vi "MQTT Client - Read.vi"(0 "MQTT Session":T2, 7 "timeout (global)":i32=10, 11 "error in (no error)":errorcluster) -> (2 "# received":u64, 4 "MQTT Session out":T2, 6 "Topic":string, 8 "Message":string, 10 "New message?":bool, 14 "Publish Properties Received (V5)":T1[](array[typedef]) {"Property" items=[" Payload Format Indicator          "=1, " Message Expiry Interval           "=2, " Content Type                      "=3, " Response Topic                    "=8, " Correlation Data                  "=9, " Subscription Identifier           "=11, " Topic Alias                       "=35, " User Property                     "=38]}, 15 "error out":errorcluster)   [LabVIEW 2019, in "KoRE-MQTT.lvlib"]
doc: "<b>Description:</b> This VI manages the core reading operations of the MQTT client by continuously checking for incoming messages from the broker. It handles message reception while maintaining the MQTT session, integrating Quality of Service (QoS) features, and facilitating message processing.\n\n<b>Input Terminals:</b>\n- <b>MQTT Session [0]</b>: Reference to the active MQTT session that allows communication with the broker.\n- <b>timeout (global) [7]</b>: Time interval in seconds for waiting for incoming messages before timing out.\n\n<b>Output Terminals:</b>\n- <b># received [2]</b>: Number of messages received from the broker during the execution of this VI.\n- <b>MQTT Session out [4]</b>: Reference to the active MQTT session after processing the read operation.\n- <b>Topic [6]</b>: The topic associated with the last received message, provided only when \"New message?\" is true.\n- <b>Message [8]</b>: The content of the last message that was received, provided only when \"New message?\" is true.\n- <b>New message? [10]</b>: Boolean value indicating whether a new message has been received since the last iteration. If false, no new messages are available, or the VI is busy handling subscriptions or QoS.\n- <b>Publish Properties [14]</b>: Array of properties associated with the last message received, applicable only for MQTT v5 connections, provided only when \"New message?\" is true.\n\n\nCopyright (c) 2025 KoRElibs.com\nSPDX-License-Identifier: EUPL-1.2\n\nThis VI is licensed under the European Union Public License (EUPL) Version 1.2. You may use this VI unmodified in proprietary works. If you distribute a modified version of this file, the modified file must be released under the EUPL-1.2. Full license: https://joinup.ec.europa.eu/asset/eupl/eupl/1.2/"
uses:
  KoRE-MQTT.lvlib
  TypeDefs/MQTT Client Session.ctl
  TypeDefs/MQTT Property - PUBLISH.ctl
  TypeDefs/MQTT Property Type.ctl
  Private/TypeDefs/MQTT Packet - Type.ctl
  Private/TypeDefs/MQTT Client Session - Data Value Reference.ctl
  TypeDefs/MQTT Client Session - Data.ctl
  TypeDefs/MQTT Property - Will.ctl
  TypeDefs/MQTT Property - CONNECT.ctl
  Private/TypeDefs/MQTT Subscription - Info.ctl
  Private/MQTT Session - Get TCP Info.vi
  Private/MQTT Session - Reset Keep Alive Timer.vi
  Private/MQTT Data Stream - Write Packet.vi
  Private/MQTT Data - Encode Varint.vi
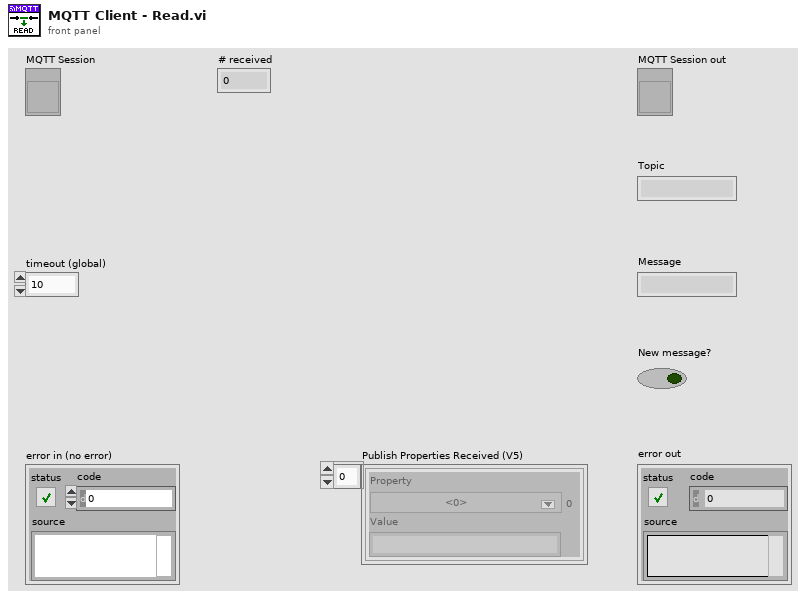
[diagram p1: front panel]
types:
  T1 = typedef "KoRE-MQTT.lvlib/MQTT Property - PUBLISH.ctl" = cluster{"Property":u8, "Value":string}
  T2 = typedef "KoRE-MQTT.lvlib/MQTT Client Session.ctl" = refnum<vi>
  T3 = typedef "KoRE-MQTT.lvlib/MQTT Packet - Type.ctl" = enum32{"Reserved", "CONNECT", "CONNACK", "PUBLISH", "PUBACK", "PUBREC", "PUBREL", "PUBCOMP", "SUBSCRIBE", "SUBACK", "UNSUBSCRIBE", "UNSUBACK", "PINGREQ", "PINGRESP", "DISCONNECT", "AUTH"}
  T4 = typedef "KoRE-MQTT.lvlib/MQTT Client Session - Data Value Reference.ctl" = refnum<data-value>
  T5 = typedef "KoRE-MQTT.lvlib/MQTT Packet - Fixed Header.ctl" = cluster{"MessageType":T3, "DUP Flag":bool, "QoS Level":u8, "RETAIN":bool, "Remaining Length":u32}
  T6 = typedef "KoRE-MQTT.lvlib/MQTT Property Type.ctl" = u8
  T7 = typedef "KoRE-MQTT.lvlib/MQTT Property - GENERIC.ctl" = cluster{"Property":T6, "Value":string}
  T8 = typedef "KoRE-MQTT.lvlib/MQTT Client Session - Data.ctl" = cluster{"TCP ref":refnum<k5>, "Next Packet Id":u16, "Version":u8, "Host":string, "Port":u16, "Ping Delta":u32, "Username":string, "Password":string, "Will QoS":u8, "Will Retain":bool, "Will Topic":string, "Will Payload":string, "TCP Timeout":i32, "Semaphore":T9, "In-Flight Messages":variant, "Close":bool, "Last Send":u32, "Keep Alive":u16, "Last Ping RTT":u32, "Last Ping":u32, "Will Properties":T10[], "Session Expiry Interval":u32, "Maximum QoS":u8, "Retain Available":bool, "Server Maximum Packet Size":u32, "Client Identifier":string, "Server Topic Alias Maximum":u16, "Wildcard Subscription Available":bool, "Subscription Identifier Available":bool, "Shared Subscription Available":bool, "Connect Properties":T11[], "Client Maximum Packet Size":u32, "Client Topic Alias Maximum":u16, "Server Receive Maximum":u16, "Client Receive Maximum":u16, "TLS cfg":refnum<k36>, "Subscriptions":T12[]}
  T9 = typedef "Semaphore RefNum" = refnum<k1>
  T10 = typedef "KoRE-MQTT.lvlib/MQTT Property - Will.ctl" = cluster{"Property":u8, "Value":string}
  T11 = typedef "KoRE-MQTT.lvlib/MQTT Property - CONNECT.ctl" = cluster{"Property":u8, "Value":string}
  T12 = typedef "KoRE-MQTT.lvlib/MQTT Subscription - Info.ctl" = cluster{"Packet Id":u16, "Index":u16, "Identifier":u32, "QoS":u8, "Topic Filter":string, "Reason Code":u8, "Reason String":string, "Granted":bool}
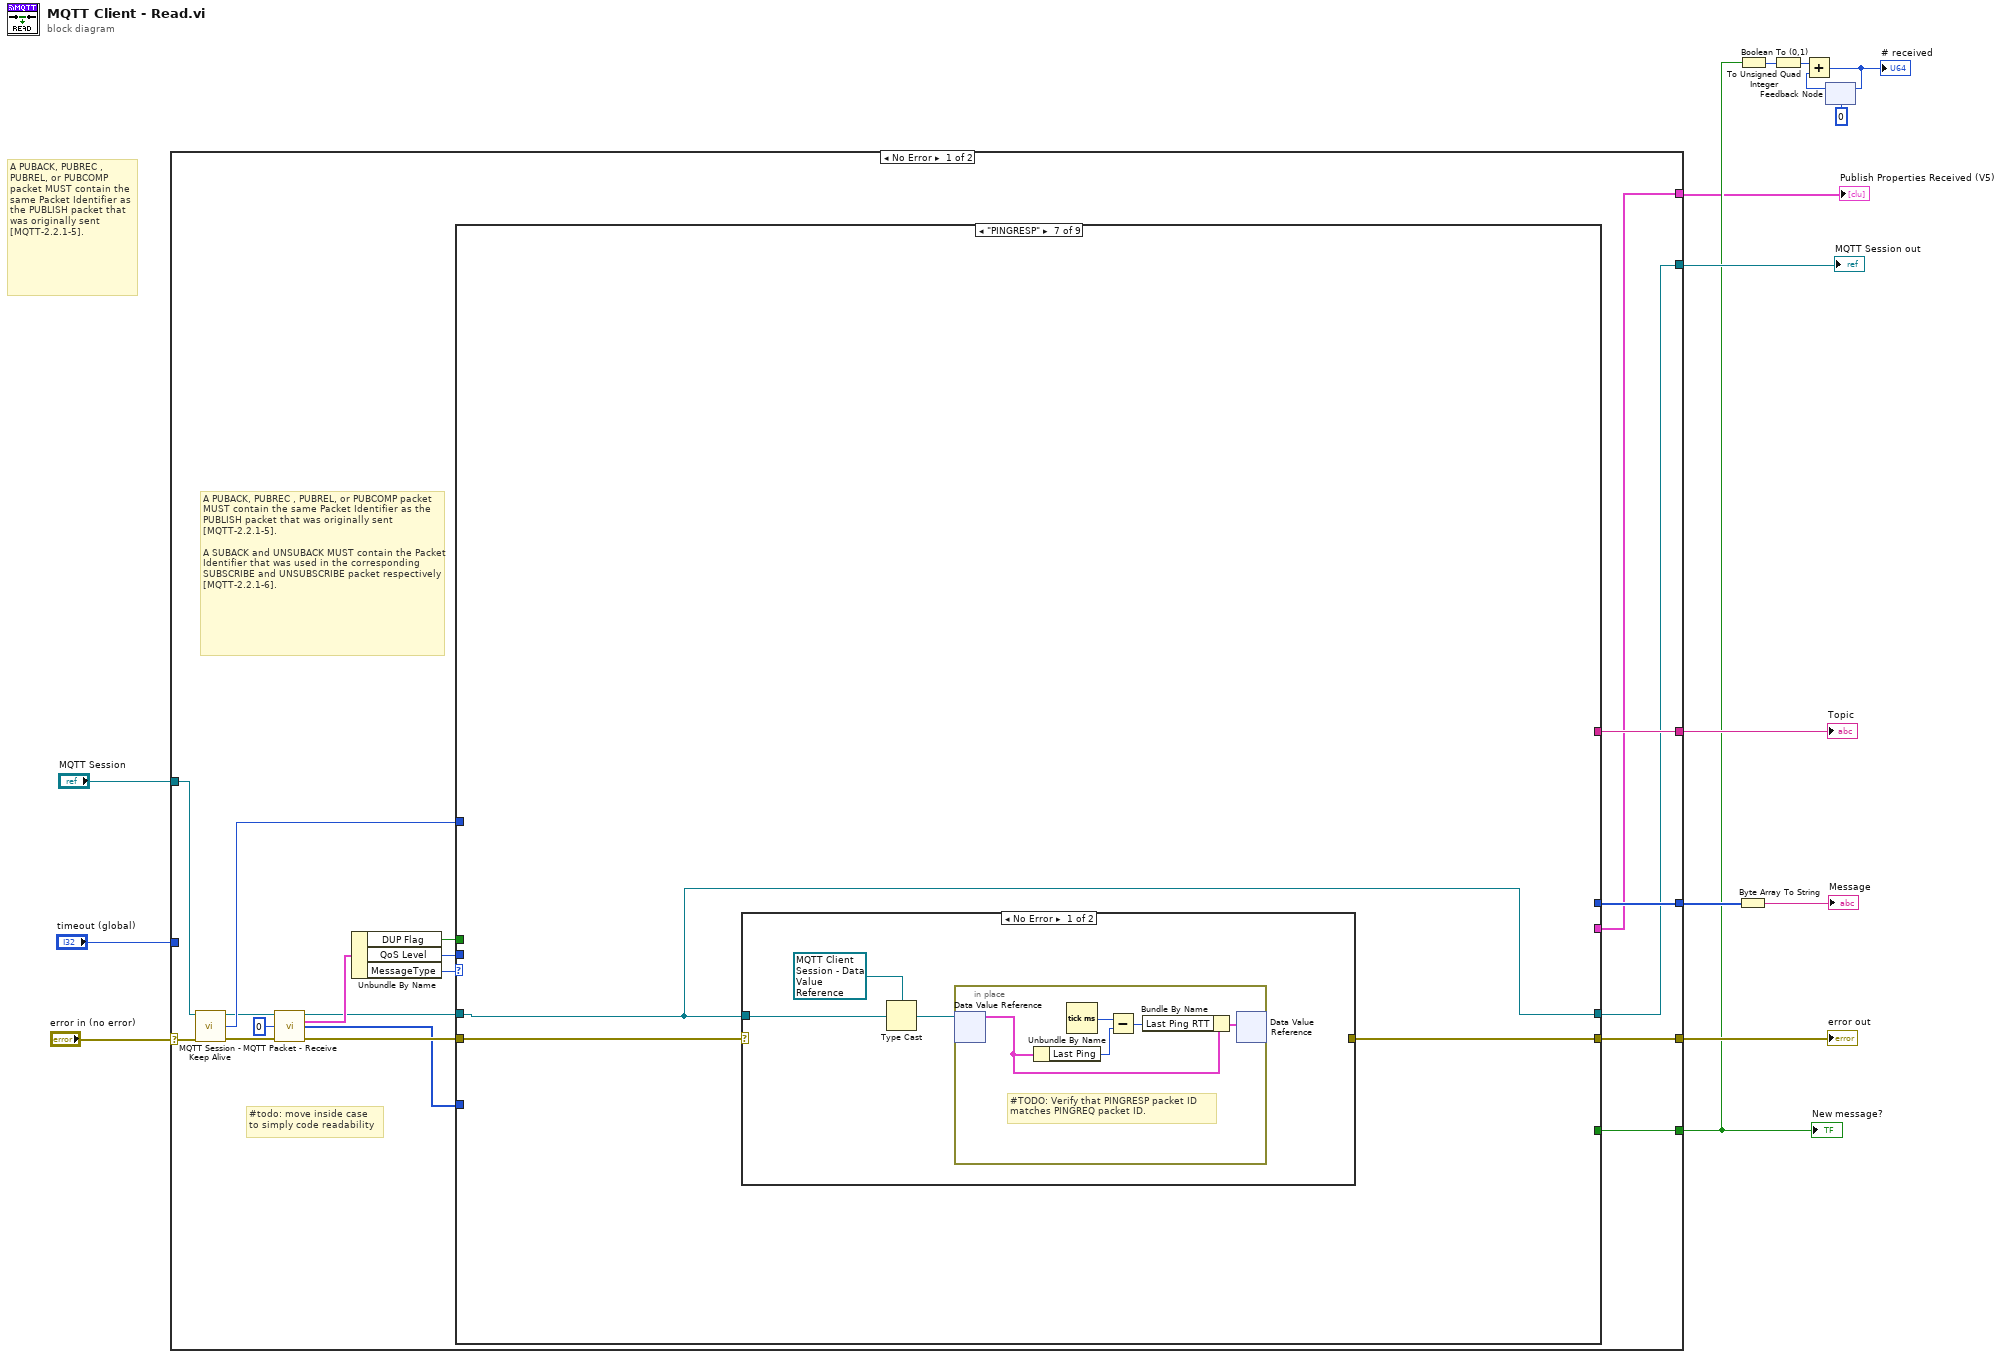
[diagram p0: block diagram]
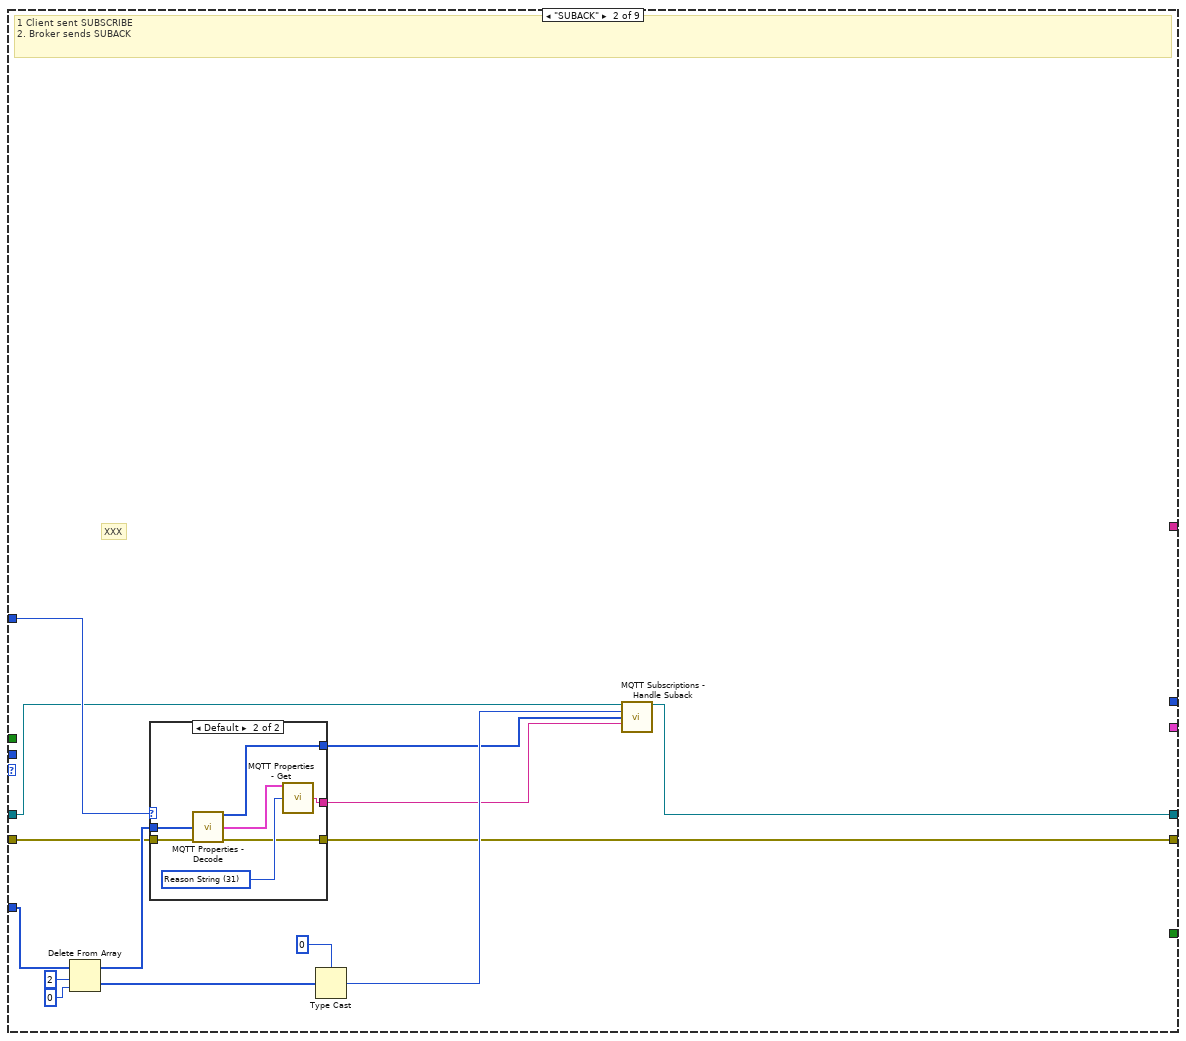
[diagram p3: hidden frame]
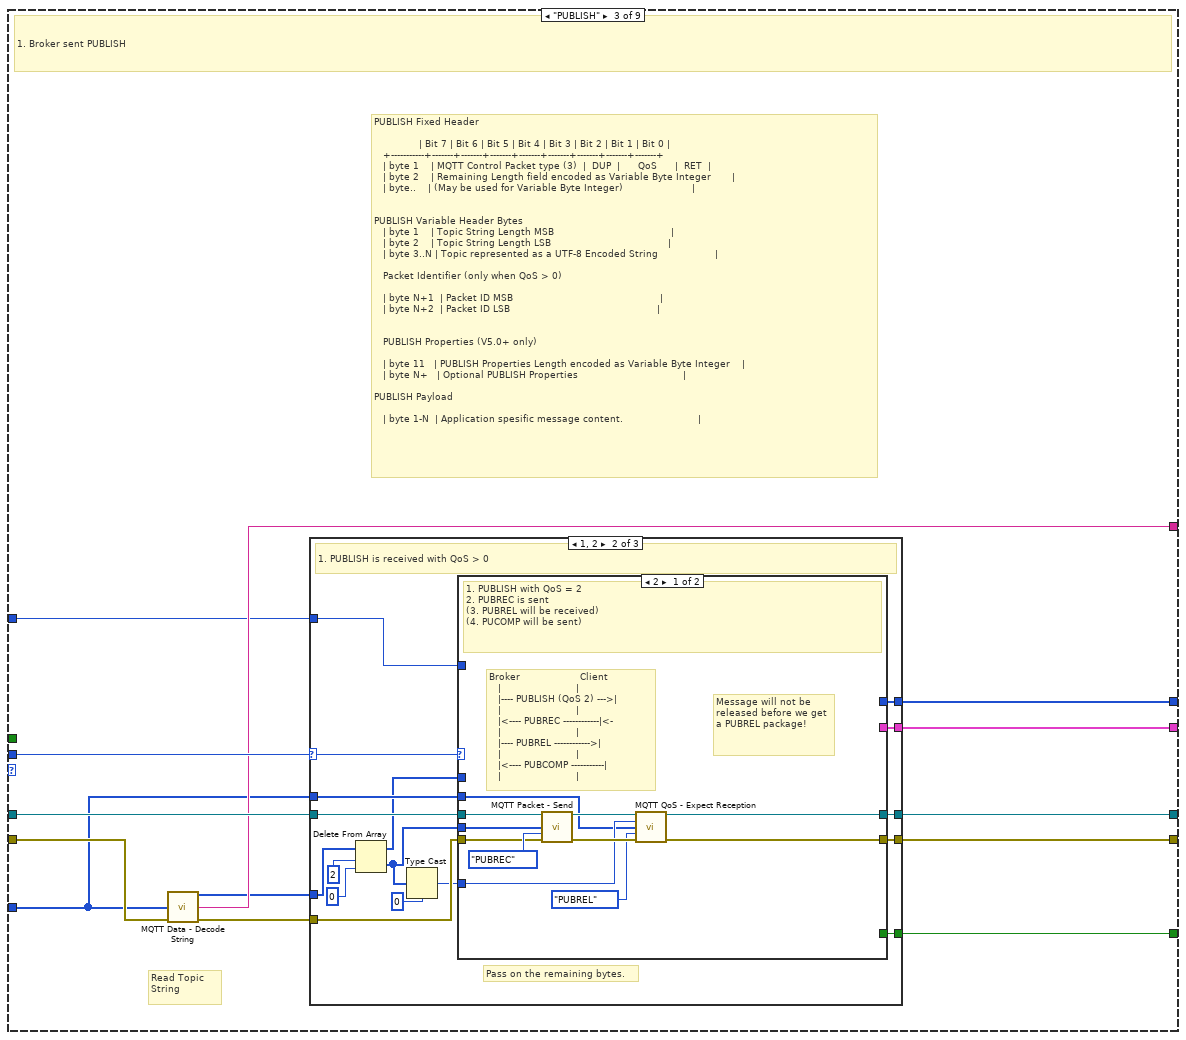
[diagram p5: hidden frame]
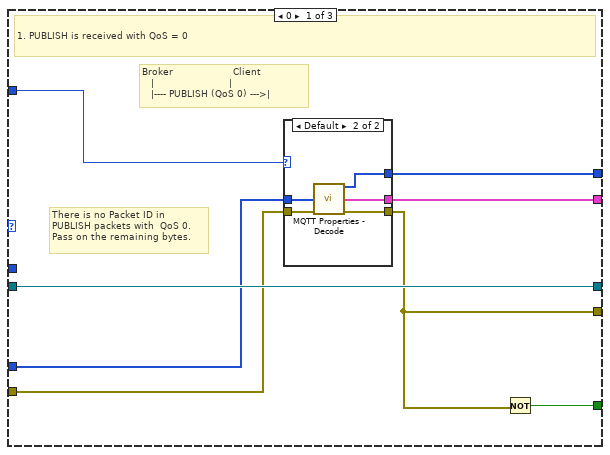
[diagram p6: hidden frame]
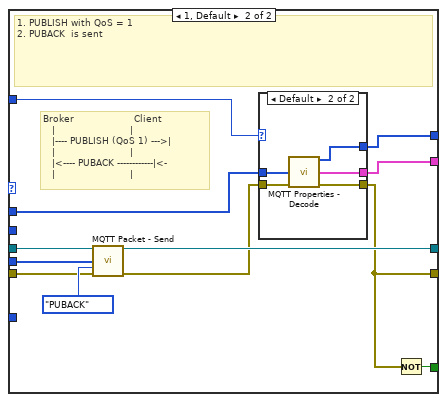
[diagram p8: hidden frame]
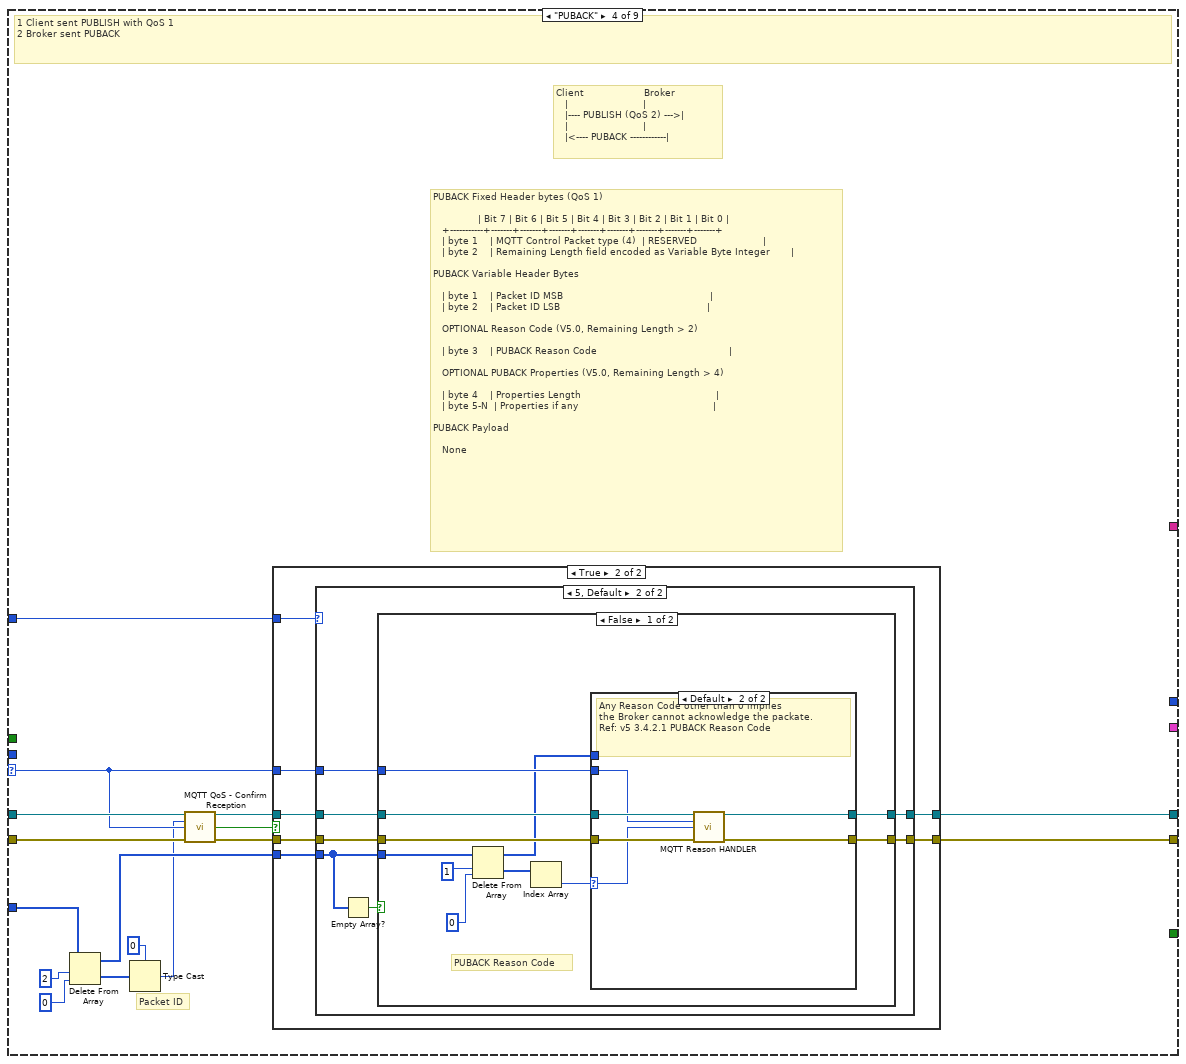
[diagram p11: hidden frame]
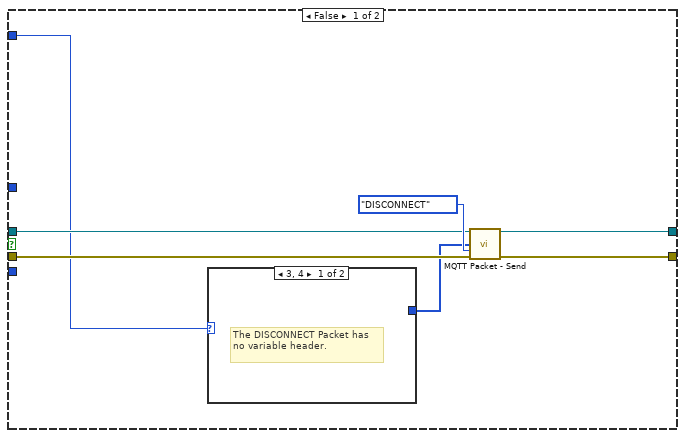
[diagram p12: hidden frame]
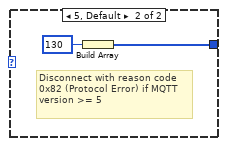
[diagram p13: hidden frame]
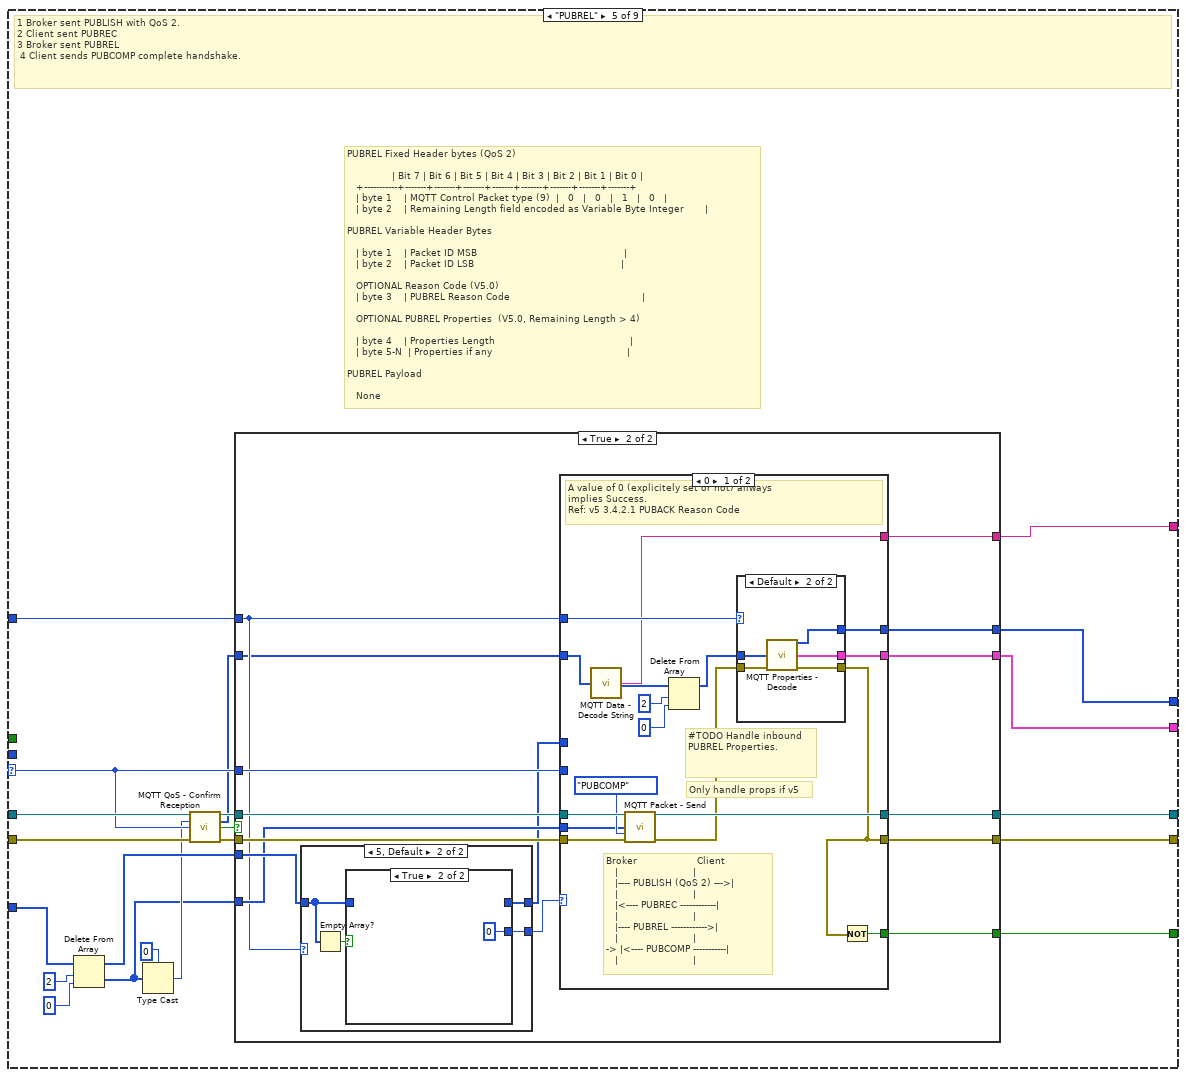
[diagram p17: hidden frame]
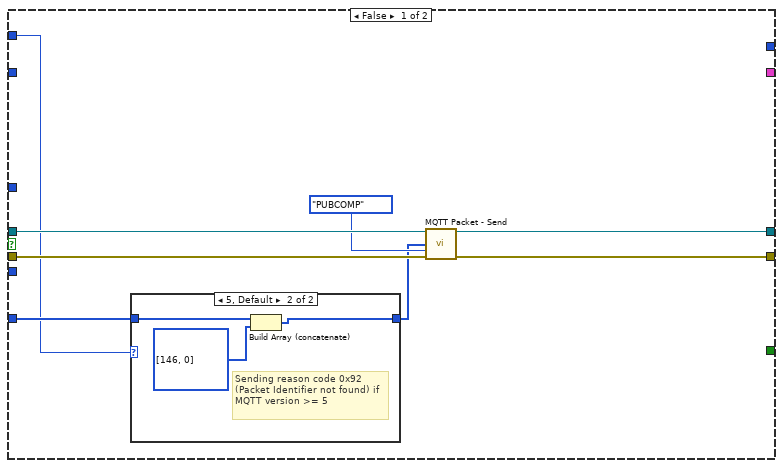
[diagram p18: hidden frame]
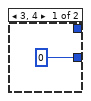
[diagram p20: hidden frame]
diagram:
  # "A PUBACK, PUBREC , PUBREL, or PUBCOMP packet MUST contain the same Packet Identifier as the PUBLISH packet that was originally sent [MQTT-2.2.1-5]."
  n1 = case shown="No Error" "error in (no error)" {
    selector: "error in (no error)" -> [w31 w387]
    tunnel: [w25 w387] -> w14
    tunnel: "MQTT Session" -> [w19 w386]
    tunnel: [w24 w386] -> w12
    tunnel: "timeout (global)" -> [_ _]
    tunnel: [w34 _] -> w10
    tunnel: [w33 _] -> w8
    tunnel: [w23 _] -> w4
    tunnel: [w21 _] -> w1
    frame No Error {
      # "#todo: move inside case \nto simply code readability"
      # "A PUBACK, PUBREC , PUBREL, or PUBCOMP packet MUST contain the same Packet Identifier as the PUBLISH packet that was originally sent [MQTT-2.2.1-5].\n\nA SUBACK and UNSUBACK MUST contain the Packet Identifier that was used in the corresponding SUBSCRIBE and UNSUBSCRIBE packet respectively [MQTT-2.2.1-6]."
      n2 = call "MQTT Session - Keep Alive.vi"("mqtt ref in"=w19, "error in"=w31) -> ("mqtt ref out"=w28:T2, "Version"=w32:u8, "error out"=w29:errorcluster)  [unwired: 11 in]
      n3 = call "MQTT Packet - Receive.vi"("mqtt ref in"=w28, "timeout (global)"=0, "error in"=w29) -> ("mqtt ref out"=w18:T2, "Fixed Header"=w30:T5, "Remaining Data"=w16:u8[], "error out"=w17:errorcluster)  [unwired: 7 in, 2 out]
      n4 = Unbundle By Name(w30) -> ("DUP Flag"=w26:bool, "QoS Level"=w27:u8, "MessageType"=w22:T3)
      n5 = case shown="\"PINGRESP\"" w22 {
        selector: w22 -> [_ _ _ w140 w207 w300 _ _ w363]
        tunnel: w27 -> [_ _ w72 _ _ _ _ _ _]
        tunnel: w32 -> [_ w50 w65 w150 w218 w294 _ w346 w364]
        tunnel: [_ _ w70 _ w198 _ _ _ _] -> w34
        tunnel: [_ _ w64 _ w201 _ _ _ _] -> w33
        tunnel: w18 -> [w36 w38 w71 w145 w213 w298 w326 w337 w368]
        tunnel: w17 -> [w35 w39 w68 w144 w211 w299 w327 w338 w369]
        tunnel: [w36 w46 w62 w152 w217 w292 w326 w347 w374] -> w24
        tunnel: [w35 w37 w61 w151 w216 w291 w325 w340 w373] -> w25
        tunnel: w26 -> [_ _ _ _ _ _ _ _ _]
        tunnel: [_ _ w66 _ w199 _ _ _ _] -> w23
        tunnel: w16 -> [_ w42 w60 w147 w208 w293 _ w343 w370]
        tunnel: [_ _ w63 _ w200 _ _ _ _] -> w21
        frame Default {
          # "#TODO:  Handle reading of unknown/unsupported MQTT Packet types, e.i. log / error handling."
        }
        frame "SUBACK" {
          # "XXX"
          # "1 Client sent SUBSCRIBE\n2. Broker sends SUBACK"
          n6 = Delete From Array(array=w42, length=2, index=0) -> (deleted portion=w40:u8[], array with subset deleted=w41:u8[])
          n7 = case shown="Default" w50 {
            tunnel: [w52 w59] -> w47
            tunnel: w41 -> [w52 w58]
            tunnel: [_ w56] -> w45
            tunnel: w39 -> [w51 w54]
            tunnel: [w51 w53] -> w37
            frame 3, 4 {
            }
            frame Default {
              w55 = T6 31 items=["Payload Format Indicator"=1, "Message Expiry Interval"=2, "Content Type"=3, "Response Topic"=8, "Correlation Data"=9, "Subscription Identifier"=11, "Session Expiry Interval"=17, "Assigned Client Identifier"=18, "Server Keep Alive"=19, "Authentication Method"=21, "Authentication Data"=22, "Request Problem Information"=23, "Will Delay Interval"=24, "Request Response Information"=25, "Response Information"=26, "Server Reference"=28, "Reason String"=31, "Receive Maximum"=33, "Topic Alias Maximum"=34, "Topic Alias"=35, "Maximum QoS"=36, "Retain Available"=37, "User Property"=38, "Maximum Packet Size"=39, "Wildcard Subscription Available"=40, "Subscription Identifier Available"=41, "Shared Subscription Available"=42] ("MQTT Property Type")
              n8 = call "MQTT Properties - Decode.vi"("Encoded MQTT Properties"=w58, "error in (no error)"=w54) -> ("remaining data"=w59:u8[], "MQTT Properties"=w57:T7[], "error out"=w53:errorcluster)  [unwired: 11 in]
              n9 = call "MQTT Properties - Get.vi"("MQTT Properties"=w57, "MQTT Property Type"=w55) -> ("Value"=w56:string)  [unwired: 11 in, 2 out]
            }
          }
          n10 = Type Cast(type=u16 0, x=w40) -> (*(type *) &x=w48:u16)
          n11 = call "MQTT Subscriptions - Handle Suback.vi"("MQTT ref in"=w38, "Packet ID"=w48, "Reason Codes"=w47, "Reason String"=w45) -> ("MQTT ref out"=w46:T2)  [unwired: 11 in]
        }
        frame "PUBLISH" {
          # "PUBLISH Fixed Header\n\n               | Bit 7 | Bit 6 | Bit 5 | Bit 4 | Bit 3 | Bit 2 | Bit 1 | Bit 0 |\n   +-----------+-------+-------+-------+-------+-------+-------+-------+-------+\n   | byte 1    | MQTT Control Packet type (3)  |  DUP  |      QoS      |  RET  |\n   | byte 2    | Remaining Length field encoded as Variable Byte Integer       |\n   | byte..    | (May be used for Variable Byte Integer)                       | \n\n\nPUBLISH Variable Header Bytes\n   | byte 1    | Topic String Length MSB                                       |  \n   | byte 2    | Topic String Length LSB                                       |  \n   | byte 3..N | Topic represented as a UTF-8 Encoded String                   |\n\n   Packet Identifier (only when QoS > 0)   \n\n   | byte N+1  | Packet ID MSB                                                 |  \n   | byte N+2  | Packet ID LSB                                                 |\n\n\n   PUBLISH Properties (V5.0+ only)\n\n   | byte 11   | PUBLISH Properties Length encoded as Variable Byte Integer    |\n   | byte N+   | Optional PUBLISH Properties                                   |\n\nPUBLISH Payload \n\n   | byte 1-N  | Application spesific message content.                         |"
          # "Read Topic String"
          # "1. Broker sent PUBLISH"
          n12 = call "MQTT Data - Decode String.vi"("Encoded String"=w60, "error in (no error)"=w68) -> ("remaining data"=w69:u8[], "String"=w70:string, "error out"=w67:errorcluster)  [unwired: 11 in]
          n13 = case shown="1, 2" w72 {
            selector: w72 -> [_ w102 _]
            tunnel: w69 -> [w78 w97 _]
            tunnel: w71 -> [w80 w101 w136]
            tunnel: w67 -> [w75 w100 w135]
            tunnel: [w73 w99 w135] -> w61
            tunnel: [w80 w98 w136] -> w62
            tunnel: [w79 w89 _] -> w66
            tunnel: [w77 w91 _] -> w64
            tunnel: [w76 w90 _] -> w63
            tunnel: w65 -> [w74 w92 _]
            tunnel: w60 -> [_ w93 _]
            frame 0 {
              # "There is no Packet ID in\nPUBLISH packets with  QoS 0.\nPass on the remaining bytes."
              # "Broker                    Client\n   |                         |\n   |---- PUBLISH (QoS 0) --->|"
              # "1. PUBLISH is received with QoS = 0"
              n14 = case shown="Default" w74 {
                tunnel: w78 -> [w82 w87]
                tunnel: [w82 w86] -> w77
                tunnel: [_ w85] -> w76
                tunnel: w75 -> [w81 w84]
                tunnel: [w81 w83] -> w73
                frame 3, 4 {
                }
                frame Default {
                  n15 = call "MQTT Properties - Decode.vi"("Encoded MQTT Properties"=w87, "error in (no error)"=w84) -> ("remaining data"=w86:u8[], "MQTT Properties"=w85:T7[], "error out"=w83:errorcluster)  [unwired: 11 in]
                }
              }
              n16 = Not(x=w73) -> (.not. x?=w79:bool)
            }
            frame 1, 2 {
              # "Pass on the remaining bytes."
              # "1. PUBLISH is received with QoS > 0"
              n17 = Delete From Array(array=w97, length=2, index=0) -> (deleted portion=w94:u8[], array with subset deleted=w88:u8[])
              n18 = Type Cast(type=u16 0, x=w94) -> (*(type *) &x=w95:u16)
              n19 = case shown="2" w102 {
                tunnel: w95 -> [w108 _]
                tunnel: w101 -> [w114 w126]
                tunnel: [w109 w125] -> w98
                tunnel: w100 -> [w113 w124]
                tunnel: [w111 w117] -> w99
                tunnel: w94 -> [w106 w123]
                tunnel: w93 -> [w105 _]
                tunnel: w92 -> [_ w122]
                tunnel: [_ w121] -> w91
                tunnel: [_ w119] -> w90
                tunnel: [_ w118] -> w89
                tunnel: w88 -> [_ w116]
                frame 2 {
                  # "Message will not be released before we get a PUBREL package!"
                  # "Broker                    Client\n   |                         |\n   |---- PUBLISH (QoS 2) --->|\n   |                         |\n   |<---- PUBREC ------------|<-\n   |                         |\n   |---- PUBREL ------------>|\n   |                         |\n   |<---- PUBCOMP -----------|\n   |                         |"
                  # "1. PUBLISH with QoS = 2\n2. PUBREC is sent\n(3. PUBREL will be received)\n(4. PUCOMP will be sent)"
                  n20 = call "MQTT Packet - Send.vi"("mqtt ref in"=w114, "packet data"=w106, "MessageType"=MQTT_Packet_-_Type."PUBREC", "error in (no error)"=w113) -> ("mqtt ref out"=w110:T2, "error out"=w112:errorcluster)  [unwired: 9 in, 1 out]
                  n21 = call "MQTT QoS - Expect Reception.vi"("MQTT Reference"=w110, "Packet ID"=w108, "Message"=w105, "MessageType"=MQTT_Packet_-_Type."PUBREL", "Error In"=w112) -> ("MQTT Reference"=w109:T2, "Error Out"=w111:errorcluster)  [unwired: 8 in, 1 out]
                }
                frame 1, Default {
                  # "Broker                    Client\n   |                         |\n   |---- PUBLISH (QoS 1) --->|\n   |                         |\n   |<---- PUBACK ------------|<-\n   |                         |"
                  # "1. PUBLISH with QoS = 1\n2. PUBACK  is sent"
                  n22 = call "MQTT Packet - Send.vi"("mqtt ref in"=w126, "packet data"=w123, "MessageType"=MQTT_Packet_-_Type."PUBACK", "error in (no error)"=w124) -> ("mqtt ref out"=w125:T2, "error out"=w120:errorcluster)  [unwired: 9 in, 1 out]
                  n23 = case shown="Default" w122 {
                    tunnel: w116 -> [w129 w134]
                    tunnel: [w129 w133] -> w121
                    tunnel: [_ w132] -> w119
                    tunnel: w120 -> [w128 w131]
                    tunnel: [w128 w130] -> w117
                    frame 3, 4 {
                    }
                    frame Default {
                      n24 = call "MQTT Properties - Decode.vi"("Encoded MQTT Properties"=w134, "error in (no error)"=w131) -> ("remaining data"=w133:u8[], "MQTT Properties"=w132:T7[], "error out"=w130:errorcluster)  [unwired: 11 in]
                    }
                  }
                  n25 = Not(x=w117) -> (.not. x?=w118:bool)
                }
              }
            }
            frame Default {
              # "#TODO: Handle QoS > 2. I.e. log/error."
              # "1. PUBLISH is received with QoS > 2"
            }
          }
        }
        frame "PUBACK" {
          # "Packet ID"
          # "PUBACK Fixed Header bytes (QoS 1)\n\n               | Bit 7 | Bit 6 | Bit 5 | Bit 4 | Bit 3 | Bit 2 | Bit 1 | Bit 0 |\n   +-----------+-------+-------+-------+-------+-------+-------+-------+-------+\n   | byte 1    | MQTT Control Packet type (4)  | RESERVED                      |\n   | byte 2    | Remaining Length field encoded as Variable Byte Integer       |\n\nPUBACK Variable Header Bytes\n\n   | byte 1    | Packet ID MSB                                                 |  \n   | byte 2    | Packet ID LSB                                                 |\n\n   OPTIONAL Reason Code (V5.0, Remaining Length > 2)\n\n   | byte 3    | PUBACK Reason Code                                            |\n\n   OPTIONAL PUBACK Properties (V5.0, Remaining Length > 4)\n\n   | byte 4    | Properties Length                                             |\n   | byte 5-N  | Properties if any                                             |\n\nPUBACK Payload\n\n   None"
          # "Client                    Broker\n   |                         |\n   |---- PUBLISH (QoS 2) --->|\n   |                         |\n   |<---- PUBACK ------------|"
          # "1 Client sent PUBLISH with QoS 1\n2 Broker sent PUBACK"
          n26 = Delete From Array(array=w147, length=2, index=0) -> (deleted portion=w138:u8[], array with subset deleted=w146:u8[])
          n27 = Type Cast(type=u16 0, x=w138) -> (*(type *) &x=w137:u16)
          n28 = call "MQTT QoS - Confirm Reception.vi"("MQTT Reference"=w145, "PacketID"=w137, "MessageType"=w140, "Error In"=w144) -> ("MQTT Reference"=w141:T2, "Found?"=w143:bool, "Error Out"=w142:errorcluster)  [unwired: 8 in, 1 out]
          n29 = case shown="True" w143 {
            tunnel: w142 -> [w156 w168]
            tunnel: w141 -> [w155 w167]
            tunnel: w140 -> [_ w166]
            tunnel: [w158 w165] -> w152
            tunnel: [w157 w164] -> w151
            tunnel: w146 -> [_ w163]
            tunnel: w150 -> [w154 w162]
            frame False {
              n30 = case shown="3, 4" w154 {
                tunnel: [_ w160] -> w153
                frame 3, 4 {
                  # "The DISCONNECT Packet has no variable header."
                }
                frame 5, Default {
                  # "Disconnect with reason code 0x82 (Protocol Error) if MQTT version >= 5"
                  n31 = Build Array(u8 130 ("Numeric")) -> (w160:u8[])
                }
              }
              n32 = call "MQTT Packet - Send.vi"("mqtt ref in"=w155, "packet data"=w153, "MessageType"=MQTT_Packet_-_Type."DISCONNECT", "error in (no error)"=w156) -> ("mqtt ref out"=w158:T2, "error out"=w157:errorcluster)  [unwired: 9 in, 1 out]
            }
            frame True {
              n33 = case shown="5, Default" w162 {
                tunnel: w168 -> [w170 w177]
                tunnel: w167 -> [w169 w176]
                tunnel: w166 -> [_ w175]
                tunnel: [w169 w174] -> w165
                tunnel: [w170 w173] -> w164
                tunnel: w163 -> [_ w172]
                frame 3, 4 {
                }
                frame 5, Default {
                  n34 = Empty Array?(array=w172) -> (empty?=w171:bool)
                  n35 = case shown="False" w171 {
                    tunnel: w177 -> [w188 w197]
                    tunnel: w176 -> [w187 w196]
                    tunnel: w175 -> [w186 _]
                    tunnel: [w185 w196] -> w174
                    tunnel: [w184 w197] -> w173
                    tunnel: w172 -> [w179 _]
                    frame False {
                      # "PUBACK Reason Code"
                      n36 = Delete From Array(array=w179, length=1, index=0) -> (deleted portion=w181:u8[], array with subset deleted=w178:u8[])
                      n37 = Index Array(array=w181) -> (element=w180:u8)  [unwired: 1 in]
                      n38 = case shown="Default" w180 {
                        selector: w180 -> [_ w191]
                        tunnel: w188 -> [w190 w193]
                        tunnel: [w190 w192] -> w184
                        tunnel: w187 -> [w189 w195]
                        tunnel: [w189 w195] -> w185
                        tunnel: w186 -> [_ w194]
                        tunnel: w178 -> [_ _]
                        frame 0 {
                          # "#TODO Handle inbound PUBACK Properties"
                          # "A value of 0 (explicitely set or not) allways\nimplies Success.\nRef: v5 3.4.2.1 PUBACK Reason Code"
                        }
                        frame Default {
                          # "Any Reason Code other than 0 implies\nthe Broker cannot acknowledge the packate.\nRef: v5 3.4.2.1 PUBACK Reason Code"
                          n39 = call "MQTT Reason HANDLER.vi"("MessageType"=w194, "Reason Code"=w191, "error in (no error)"=w193) -> ("error out"=w192:errorcluster)  [unwired: 12 in]
                        }
                      }
                    }
                    frame True {
                    }
                  }
                }
              }
            }
          }
        }
        frame "PUBREL" {
          # "PUBREL Fixed Header bytes (QoS 2)\n\n               | Bit 7 | Bit 6 | Bit 5 | Bit 4 | Bit 3 | Bit 2 | Bit 1 | Bit 0 |\n   +-----------+-------+-------+-------+-------+-------+-------+-------+-------+\n   | byte 1    | MQTT Control Packet type (9)  |   0   |   0   |   1   |   0   |\n   | byte 2    | Remaining Length field encoded as Variable Byte Integer       |\n\nPUBREL Variable Header Bytes\n\n   | byte 1    | Packet ID MSB                                                 |  \n   | byte 2    | Packet ID LSB                                                 |\n\n   OPTIONAL Reason Code (V5.0) \n   | byte 3    | PUBREL Reason Code                                            |\n\n   OPTIONAL PUBREL Properties  (V5.0, Remaining Length > 4)\n\n   | byte 4    | Properties Length                                             |\n   | byte 5-N  | Properties if any                                             |\n                 \nPUBREL Payload\n\n   None"
          # "1 Broker sent PUBLISH with QoS 2.\n2 Client sent PUBREC\n3 Broker sent PUBREL\n 4 Client sends PUBCOMP complete handshake."
          n40 = Delete From Array(array=w208, length=2, index=0) -> (deleted portion=w203:u8[], array with subset deleted=w209:u8[])
          n41 = Type Cast(type=u16 0, x=w203) -> (*(type *) &x=w204:u16)
          n42 = call "MQTT QoS - Confirm Reception.vi"("MQTT Reference"=w213, "PacketID"=w204, "MessageType"=w207, "Error In"=w211) -> ("MQTT Reference"=w212:T2, "Released Message"=w202:u8[], "Found?"=w206:bool, "Error Out"=w210:errorcluster)  [unwired: 8 in]
          n43 = case shown="True" w206 {
            tunnel: w210 -> [w226 w245]
            tunnel: w212 -> [w223 w244]
            tunnel: w207 -> [_ w243]
            tunnel: [w224 w242] -> w217
            tunnel: [w225 w241] -> w216
            tunnel: w209 -> [_ w240]
            tunnel: w218 -> [w220 w236]
            tunnel: w203 -> [w222 w239]
            tunnel: w202 -> [_ w235]
            tunnel: [_ w234] -> w201
            tunnel: [_ w233] -> w200
            tunnel: [_ w232] -> w199
            tunnel: [_ w231] -> w198
            frame False {
              n44 = case shown="5, Default" w220 {
                tunnel: w222 -> [w227 w230]
                tunnel: [w227 w229] -> w219
                frame 3, 4 {
                }
                frame 5, Default {
                  # "Sending reason code 0x92 (Packet Identifier not found) if MQTT version >= 5"
                  n45 = Build Array (concatenate)(w230, u8[] [146, 0] ("payload")) -> (w229:u8[])
                }
              }
              n46 = call "MQTT Packet - Send.vi"("mqtt ref in"=w223, "packet data"=w219, "MessageType"=MQTT_Packet_-_Type."PUBCOMP", "error in (no error)"=w226) -> ("mqtt ref out"=w224:T2, "error out"=w225:errorcluster)  [unwired: 9 in, 1 out]
            }
            frame True {
              n47 = case shown="5, Default" w236 {
                tunnel: w240 -> [_ w247]
                tunnel: [u8 0 w250] -> w238
                tunnel: [_ w249] -> w237
                frame 3, 4 {
                }
                frame 5, Default {
                  n48 = Empty Array?(array=w247) -> (empty?=w248:bool)
                  n49 = case shown="True" w248 {
                    tunnel: w247 -> [w256 _]
                    tunnel: [w252 u8 0] -> w250
                    tunnel: [w251 _] -> w249
                    frame False {
                      # "PUBREL Reason Code"
                      n50 = Delete From Array(array=w256, length=1, index=0) -> (deleted portion=w253:u8[], array with subset deleted=w251:u8[])
                      n51 = Index Array(array=w253) -> (element=w252:u8)  [unwired: 1 in]
                    }
                    frame True {
                    }
                  }
                }
              }
              n52 = case shown="0" w238 {
                selector: w238 -> [_ w282]
                tunnel: w245 -> [w274 w284]
                tunnel: [w265 w283] -> w241
                tunnel: w244 -> [w273 w286]
                tunnel: [w272 w286] -> w242
                tunnel: w243 -> [_ w285]
                tunnel: w239 -> [w270 _]
                tunnel: w237 -> [_ _]
                tunnel: w236 -> [w269 _]
                tunnel: w235 -> [w263 _]
                tunnel: [w267 _] -> w234
                tunnel: [w266 _] -> w233
                tunnel: [w264 _] -> w232
                tunnel: [w262 _] -> w231
                frame 0 {
                  # "Only handle props if v5"
                  # "#TODO Handle inbound PUBREL Properties."
                  # "Broker                    Client\n   |                         |\n   |---- PUBLISH (QoS 2) --->|\n   |                         |\n   |<---- PUBREC ------------|\n   |                         |\n   |---- PUBREL ------------>|\n   |                         |\n-> |<---- PUBCOMP -----------|\n   |                         |"
                  # "A value of 0 (explicitely set or not) allways\nimplies Success.\nRef: v5 3.4.2.1 PUBACK Reason Code"
                  n53 = call "MQTT Data - Decode String.vi"("Encoded String"=w263) -> ("remaining data"=w259:u8[], "String"=w262:string)  [unwired: 12 in, 1 out]
                  n54 = call "MQTT Packet - Send.vi"("mqtt ref in"=w273, "packet data"=w270, "MessageType"=MQTT_Packet_-_Type."PUBCOMP", "error in (no error)"=w274) -> ("mqtt ref out"=w272:T2, "error out"=w268:errorcluster)  [unwired: 9 in, 1 out]
                  n55 = Delete From Array(array=w259, length=2, index=0) -> (array with subset deleted=w258:u8[])  [unwired: 1 out]
                  n56 = case shown="Default" w269 {
                    tunnel: w258 -> [w276 w281]
                    tunnel: [w276 w280] -> w267
                    tunnel: [_ w279] -> w266
                    tunnel: w268 -> [w275 w278]
                    tunnel: [w275 w277] -> w265
                    frame 3, 4 {
                    }
                    frame Default {
                      n57 = call "MQTT Properties - Decode.vi"("Encoded MQTT Properties"=w281, "error in (no error)"=w278) -> ("remaining data"=w280:u8[], "MQTT Properties"=w279:T7[], "error out"=w277:errorcluster)  [unwired: 11 in]
                    }
                  }
                  n58 = Not(x=w265) -> (.not. x?=w264:bool)
                }
                frame Default {
                  # "Any Reason Code other than 0 implies\nthe Broker cannot acknowledge the packate.\nRef: v5 3.4.2.1 PUBREL Reason Code"
                  n59 = call "MQTT Reason HANDLER.vi"("MessageType"=w285, "Reason Code"=w282, "error in (no error)"=w284) -> ("error out"=w283:errorcluster)  [unwired: 12 in]
                }
              }
            }
          }
        }
        frame "PUBREC" {
          # "PUBREL Fixed Header bytes (QoS 2)\n\n               | Bit 7 | Bit 6 | Bit 5 | Bit 4 | Bit 3 | Bit 2 | Bit 1 | Bit 0 |\n   +-----------+-------+-------+-------+-------+-------+-------+-------+-------+\n   | byte 1    | MQTT Control Packet type (9)  |   0   |   0   |   1   |   0   |\n   | byte 2    | Remaining Length field encoded as Variable Byte Integer       |\n\nPUBREL Variable Header Bytes\n\n   | byte 1    | Packet ID MSB                                                 |  \n   | byte 2    | Packet ID LSB                                                 |\n\n   OPTIONAL Reason Code (V5.0) \n   | byte 3    | PUBREL Reason Code                                            |\n\n   OPTIONAL PUBREL Properties  (V5.0, Remaining Length > 4)\n\n   | byte 4    | Properties Length                                             |\n   | byte 5-N  | Properties if any                                             |\n                 \nPUBREL Payload\n\n   None"
          # "Packet ID"
          # "PUBREC Fixed Header bytes (QoS 2)\n\n               | Bit 7 | Bit 6 | Bit 5 | Bit 4 | Bit 3 | Bit 2 | Bit 1 | Bit 0 |\n   +-----------+-------+-------+-------+-------+-------+-------+-------+-------+\n   | byte 1    | MQTT Control Packet type (5)  | RESERVED                      |\n   | byte 2    | Remaining Length field encoded as Variable Byte Integer       |\n\nPUBREC Variable Header Bytes\n\n   | byte 1    | Packet ID MSB                                                 |  \n   | byte 2    | Packet ID LSB                                                 |\n\n   OPTIONAL Reason Code (Remaining Lengh > 2)\n\n   | byte 3    | PUBACK Reason Code                                            |\n\n   OPTIONAL PUBREC Properties (V5.0, Remaining Length > 4)\n\n   | byte 4    | Properties Length                                             |\n   | byte 5-N  | Properties if any                                             |\n\nPUBREC Payload\n\n   None"
          # "1. Client sent PUBLISH with QoS 2.\n2. Broker sends PUREC\n3. Client sends PUBREL\n(4. Broker will send PUBCOMP)"
          n60 = Delete From Array(array=w293, length=2, index=0) -> (deleted portion=w288:u8[], array with subset deleted=w290:u8[])
          n61 = Type Cast(type=u16 0, x=w288) -> (*(type *) &x=w287:u16)
          n62 = call "MQTT QoS - Confirm Reception.vi"("MQTT Reference"=w298, "PacketID"=w287, "MessageType"=w300, "Error In"=w299) -> ("MQTT Reference"=w296:T2, "Found?"=w297:bool, "Error Out"=w295:errorcluster)  [unwired: 8 in, 1 out]
          n63 = case shown="True" w297 {
            tunnel: w296 -> [w309 w319]
            tunnel: w295 -> [w308 w318]
            tunnel: w294 -> [w307 _]
            tunnel: w288 -> [w306 w315]
            tunnel: [w305 w321] -> w292
            tunnel: [w304 w320] -> w291
            tunnel: w290 -> [_ _]
            tunnel: w287 -> [_ w317]
            frame False {
              n64 = case shown="5, Default" w307 {
                tunnel: w306 -> [w311 w314]
                tunnel: [w311 w313] -> w303
                frame 3, 4 {
                }
                frame 5, Default {
                  # "Sending reason code 0x92 (Packet Identifier not found) if MQTT version >= 5"
                  n65 = Build Array (concatenate)(w314, u8[] [146, 0] ("payload")) -> (w313:u8[])
                }
              }
              n66 = call "MQTT Packet - Send.vi"("mqtt ref in"=w309, "packet data"=w303, "MessageType"=MQTT_Packet_-_Type."PUBREL", "error in (no error)"=w308) -> ("mqtt ref out"=w305:T2, "error out"=w304:errorcluster)  [unwired: 9 in, 1 out]
            }
            frame True {
              # "#TODO Handle PUBREC Properties from Broker?"
              # "Expect PUBCOMP from broker."
              # "Send PUBREL to broker."
              n67 = call "MQTT Packet - Send.vi"("mqtt ref in"=w319, "packet data"=w315, "MessageType"=MQTT_Packet_-_Type."PUBREL", "error in (no error)"=w318) -> ("mqtt ref out"=w323:T2, "error out"=w324:errorcluster)  [unwired: 9 in, 1 out]
              n68 = call "MQTT QoS - Expect Reception.vi"("MQTT Reference"=w323, "Packet ID"=w317, "Message"=w315, "MessageType"=MQTT_Packet_-_Type."PUBCOMP", "Error In"=w324) -> ("MQTT Reference"=w321:T2, "Error Out"=w320:errorcluster)  [unwired: 8 in, 1 out]
            }
          }
        }
        frame "PINGRESP" {
          n69 = case shown="No Error" w327 {
            selector: w327 -> [_ w336]
            tunnel: w326 -> [w328 _]
            tunnel: [_ w336] -> w325
            frame No Error {
              n70 = Type Cast(type=T4 refnum ("data value reference"), x=w328) -> (*(type *) &x=w329:T4)
              n71 = in-place "In Place Element Structure" {
                # "#TODO: Verify that PINGRESP packet ID\nmatches PINGREQ packet ID."
                n72 = in-place-dvr #1(w329) -> (w332:T8)  [unwired: 1 out]
                n73 = Unbundle By Name(w332) -> ("Last Ping"=w334:u32)
                n74 = Tick Count (ms)() -> (millisecond timer value=w333:u32)
                n75 = Subtract(x=w333, y=w334) -> (x-y=w335:u32)
                n76 = Bundle By Name(cluster=w332, "Last Ping RTT"=w335) -> (w331:T8)
                n77 = in-place-dvr #1(w331) -> ()  [unwired: 2 out]
              }
            }
            frame Error {
            }
          }
        }
        frame "UNSUBACK" {
          # "#todo:"
          # "#todo: store subscriptions in memory during subs\n(packet id, index, (identifier), qos, subscription filter\n\nand update here\nreason code and reason string\n\nconsider using both requested qos and actual and granted"
          # "1 Client sent UNSUBSCRIBE\n2. Broker sends UNSUBACK"
          n78 = Delete From Array(array=w343, length=2, index=0) -> (deleted portion=w341:u8[], array with subset deleted=w342:u8[])
          n79 = Type Cast(type=u16 0, x=w341) -> (*(type *) &x=w339:u16)
          n80 = case shown="5, Default" w346 {
            tunnel: [w352 w359] -> w349
            tunnel: w342 -> [w352 w358]
            tunnel: [_ w356] -> w348
            tunnel: w338 -> [w351 w354]
            tunnel: [w351 w353] -> w340
            frame 3, 4 {
            }
            frame 5, Default {
              w355 = T6 31 items=["Payload Format Indicator"=1, "Message Expiry Interval"=2, "Content Type"=3, "Response Topic"=8, "Correlation Data"=9, "Subscription Identifier"=11, "Session Expiry Interval"=17, "Assigned Client Identifier"=18, "Server Keep Alive"=19, "Authentication Method"=21, "Authentication Data"=22, "Request Problem Information"=23, "Will Delay Interval"=24, "Request Response Information"=25, "Response Information"=26, "Server Reference"=28, "Reason String"=31, "Receive Maximum"=33, "Topic Alias Maximum"=34, "Topic Alias"=35, "Maximum QoS"=36, "Retain Available"=37, "User Property"=38, "Maximum Packet Size"=39, "Wildcard Subscription Available"=40, "Subscription Identifier Available"=41, "Shared Subscription Available"=42] ("MQTT Property Type")
              n81 = call "MQTT Properties - Decode.vi"("Encoded MQTT Properties"=w358, "error in (no error)"=w354) -> ("remaining data"=w359:u8[], "MQTT Properties"=w357:T7[], "error out"=w353:errorcluster)  [unwired: 11 in]
              n82 = call "MQTT Properties - Get.vi"("MQTT Properties"=w357, "MQTT Property Type"=w355) -> ("Value"=w356:string)  [unwired: 11 in, 2 out]
            }
          }
          n83 = call "MQTT Subscriptions - Handle Unsuback.vi"("MQTT ref in"=w337, "Packet ID"=w339, "Reason Codes"=w349, "Reason String"=w348) -> ("MQTT ref out"=w347:T2)  [unwired: 11 in]
        }
        frame "PUBCOMP" {
          # "PUBCOMP Fixed Header bytes (QoS 2)\n\n               | Bit 7 | Bit 6 | Bit 5 | Bit 4 | Bit 3 | Bit 2 | Bit 1 | Bit 0 |\n   +-----------+-------+-------+-------+-------+-------+-------+-------+-------+\n   | byte 1    | MQTT Control Packet type (7)  |   0   |   0   |   1   |   0   |\n   | byte 2    | Remaining Length field encoded as Variable Byte Integer       |\n\nPUBCOMP Variable Header Bytes\n\n   | byte 1    | Packet ID MSB                                                 |  \n   | byte 2    | Packet ID LSB                                                 |\n   | byte 3    | PUBCOMP Reason Code                                           |\n\n   OPTIONAL PUBCOMP Properties  (V5.0, Remaining Length > 4)\n\n   | byte 4    | Properties Length                                             |\n   | byte 5-N  | Properties if any                                             |\n                 \nPUBCOMP Payload\n\n   None"
          # "XXX"
          # "1. Client sent PUBLISH with QoS 2.\n2. Broker sends PUREC\n3. Client sends PUBREL\n4. Broker sends PUBCOMP"
          n84 = Delete From Array(array=w370, length=2, index=0) -> (deleted portion=w361:u8[])  [unwired: 1 out]
          n85 = Type Cast(type=u16 0, x=w361) -> (*(type *) &x=w360:u16)
          n86 = call "MQTT QoS - Confirm Reception.vi"("MQTT Reference"=w368, "PacketID"=w360, "MessageType"=w363, "Error In"=w369) -> ("MQTT Reference"=w365:T2, "Found?"=w367:bool, "Error Out"=w366:errorcluster)  [unwired: 8 in, 1 out]
          n87 = case shown="True" w367 {
            tunnel: [w379 w385] -> w374
            tunnel: w365 -> [w380 w385]
            tunnel: [w378 w384] -> w373
            tunnel: w366 -> [w377 w384]
            tunnel: w364 -> [w381 _]
            frame False {
              n88 = case shown="5, Default" w381 {
                tunnel: [_ w382] -> w375
                frame 3, 4 {
                  # "The DISCONNECT Packet has no variable header."
                }
                frame 5, Default {
                  # "Disconnect with reason code 0x82 (Protocol Error) if MQTT version >= 5"
                  n89 = Build Array(u8 130 ("Numeric")) -> (w382:u8[])
                }
              }
              n90 = call "MQTT Packet - Send.vi"("mqtt ref in"=w380, "packet data"=w375, "MessageType"=MQTT_Packet_-_Type."DISCONNECT", "error in (no error)"=w377) -> ("mqtt ref out"=w379:T2, "error out"=w378:errorcluster)  [unwired: 9 in, 1 out]
            }
            frame True {
            }
          }
        }
      }
    }
    frame Error {
    }
  }
  "error out" <- w14
  "MQTT Session out" <- w12
  "Topic" <- w10
  "New message?" <- w4
  "Publish Properties Received (V5)" <- w1
  n91 = Byte Array To String(unsigned byte array=w8) -> (string=→"Message":string)
  n92 = Boolean To (0,1)(Boolean=w4) -> (0, 1=w5:i16)
  n93 = To Unsigned Quad Integer(1:w5) -> (0:w2:u64)
  n94 = feedback #2(u64 0) -> (w6:u64)
  n95 = Add(x=w2, y=w6) -> (x+y=w3:u64)
  "# received" <- w3
  n96 = feedback-in #2(w3) -> ()
